vi "ResetMedMotor.vi"   [LabVIEW 2016]
uses:
  <vilib>/NXT/Block Support/NXT_OutputPort.ctl
  <vilib>/NXT/NXTIO Xnodes/NXTIONodeSubVIs/NXTMoveMotors.vi
  <vilib>/NXT/NXTIO Xnodes/NXTIONodeSubVIs/NXTStopMotors.vi
  <vilib>/NXT/Subs/LVHSConnector.ctl
  <vilib>/NXT/NXTIO Xnodes/AddressXNode/NXTIOAddress.xnode
  PMR_081.lvrbt
  <vilib>/NXT/NXTIO Xnodes/NXTIOXNode/NXTIO.xnode
  <vilib>/NXT/LegoClasses/BrickReference/BrickReference.lvclass
types:
  T1 = typedef "NXT_OutputPort.ctl" = u8
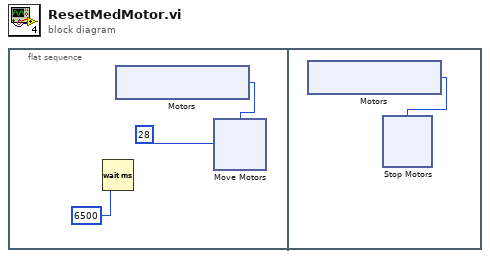
[diagram p0: block diagram]
diagram:
  n1 = flat-sequence {
    frame #0 {
      n2 = Wait (ms)(milliseconds to wait=6500) -> ()  [unwired: 1 out]
      n3 = xnode "Motors"() -> ("Motor"=w1:T1)
      n4 = xnode "Move Motors"("Power/Speed 1"=28, "Motors"=w1) -> ()  [unwired: 1 in, 1 out]
    }
    frame #1 {
      n5 = xnode "Motors"() -> ("Motor"=w12:T1)
      n6 = xnode "Stop Motors"("Motors"=w12) -> ()  [unwired: 1 in, 1 out]
    }
  }
